vi "TCP_Main.vi"() -> ()   [LabVIEW 2024]
uses:
  <vilib>/Platform/TimedLoop/XDataNode/timing_clust.ctl
  <vilib>/Platform/TimedLoop/XDataNode/nitl_modes.ctl
  <vilib>/Platform/TimedLoop/XDataNode/wakeup.ctl
  <vilib>/addons/Maxon Motor/EPOS2 CANopen/CANopen/sbCANopenBaseClass.lvclass
  <vilib>/platform/TimedLoop/XDataNode/XDataNode.xnode
  <vilib>/Platform/TimedLoop/XDataNode/XDNodeRunTimeDep.lvlib
panel:
  out "TCP Read Error":errorcluster
  out "goal_Tensions":dbl[](array[numeric])
  out "ResetPID":bool
  in  "Motor_index":i32[](array[numeric])=[3, 6, 9, 12, 2, 7, 8, 13, 4, 5, 10, 11, 1, 14]
  out "canERROR":errorcluster[][](array[cluster])
  in  "Control Mode":string="O"
  in  "TARE":bool
  in  "curr_Tensions":dbl[](array[numeric])
  out "DAQ Error":errorcluster
  out "Write Late?":bool
  out "Write Time [us]":i64
  in  "Tare_Tensions":dbl[](array[numeric])=[1.6875269817998764, 0.7228096971601798, 1.962272927280566, 2.6696462364433735, 2.7003690389898463, 3.088938448864716, 1.6430905755314908, 3.0754139877790347, 3.5546581214666455, 3.2737863413382597, 4.727265898547672, 2.6001067118162604, 1.980007529135911, 1.8614502099489874]
  in  "STOP CONTROLLER":bool
  # "\"Error\" codes:\n\n66 - Client Disconnected\n56 - TCP Read time out (every 1ms if no msg comes in)\n0 - packet received"
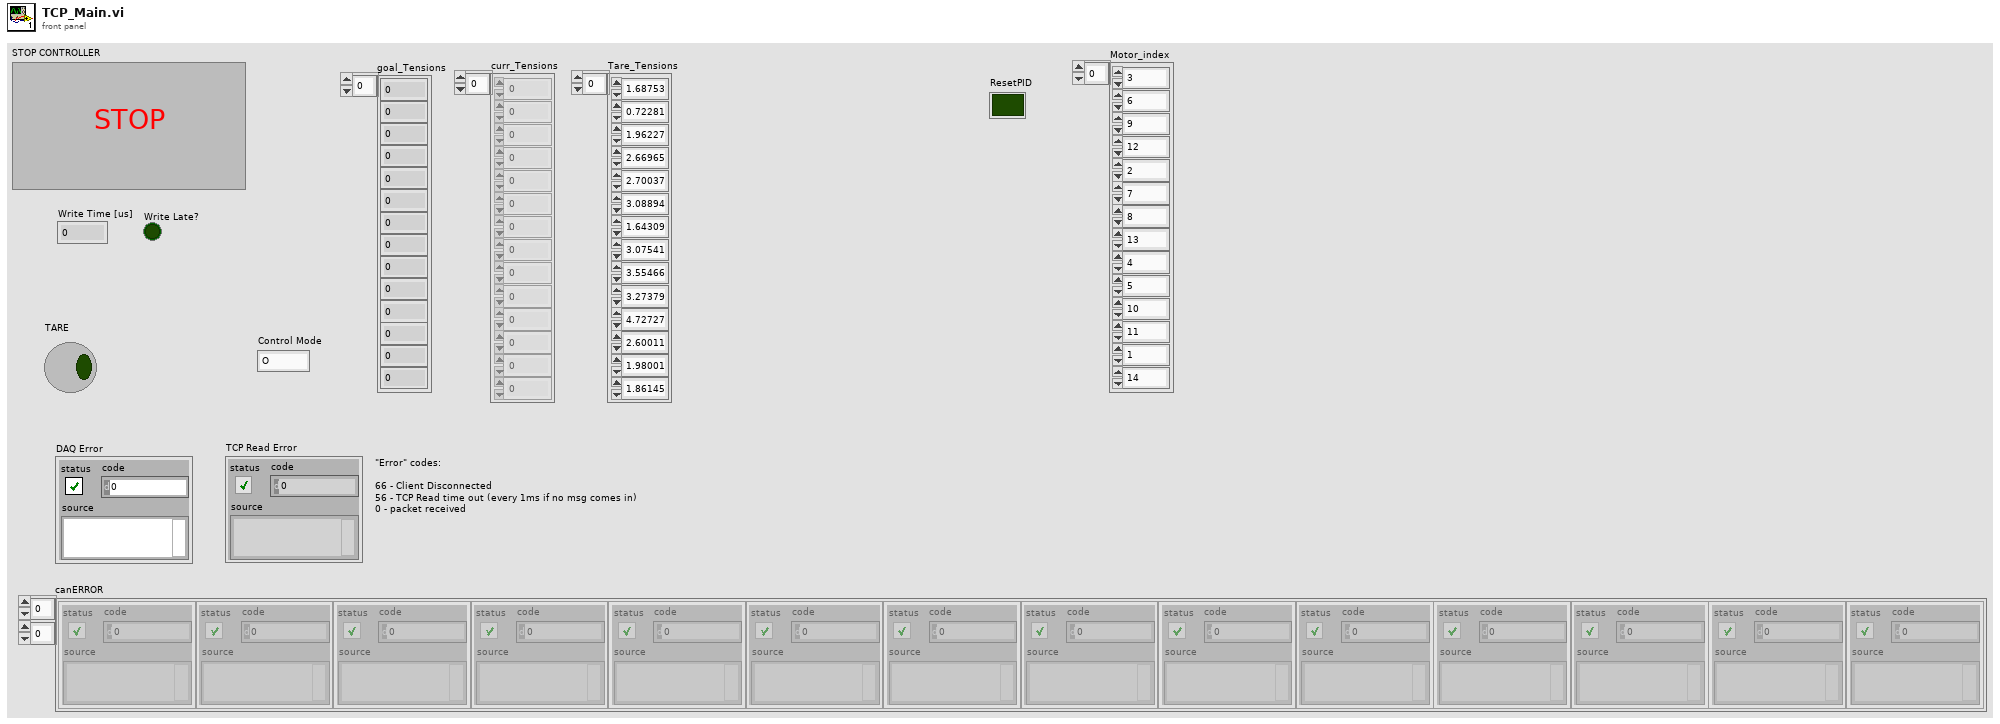
[diagram p1: front panel]
types:
  T1 = enum16{"Standard", "Buffered", "CRLF", "Immediate"}
  T2 = typedef "XDNodeRunTimeDep.lvlib/timing_clust.ctl" = cluster{"Expected End [f-1]":u64, "Actual End [f-1]":u64, "Finished Late? [f-1]":bool, "Expected End [i-1]":u64, "Actual End [i-1]":u64, "Finished Late? [i-1]":bool, "Expected Start [i]":u64, "Actual Start [i]":u64, "Expected Start [f]":u64, "Actual Start [f]":u64, "Source Name":string, "Structure Name":string, "Period":i64, "Deadline":i64, "Offset":i64, "Start":i64, "Priority":i32, "Timeout":i32, "Mode":T3, "Wakeup Reason":T4, "Error":errorcluster, "Source Type":string, "Secondary Source Type":string, "Global End Time":u64, "Global Start Time":u64, "Frame Duration":u64, "Iteration Duration":u64, "Assigned CPU":i32, "I/O Scan Engine Mode":u32}
  T3 = typedef "XDNodeRunTimeDep.lvlib/nitl_modes.ctl" = enum32{"No Change", "Process missed periods, maintain original phase", "Discard missed periods, maintain original phase", "Process missed periods, ignore original phase", "Discard missed periods, ignore original phase"}
  T4 = typedef "XDNodeRunTimeDep.lvlib/wakeup.ctl" = enum32{"Normal", "Aborted", "Asynchronous wakeup", "Timing source error", "Timed loop error", "Timeout"}
  T5 = cluster{"curr_Tensions":dbl[], "goal_Tensions":dbl[]}
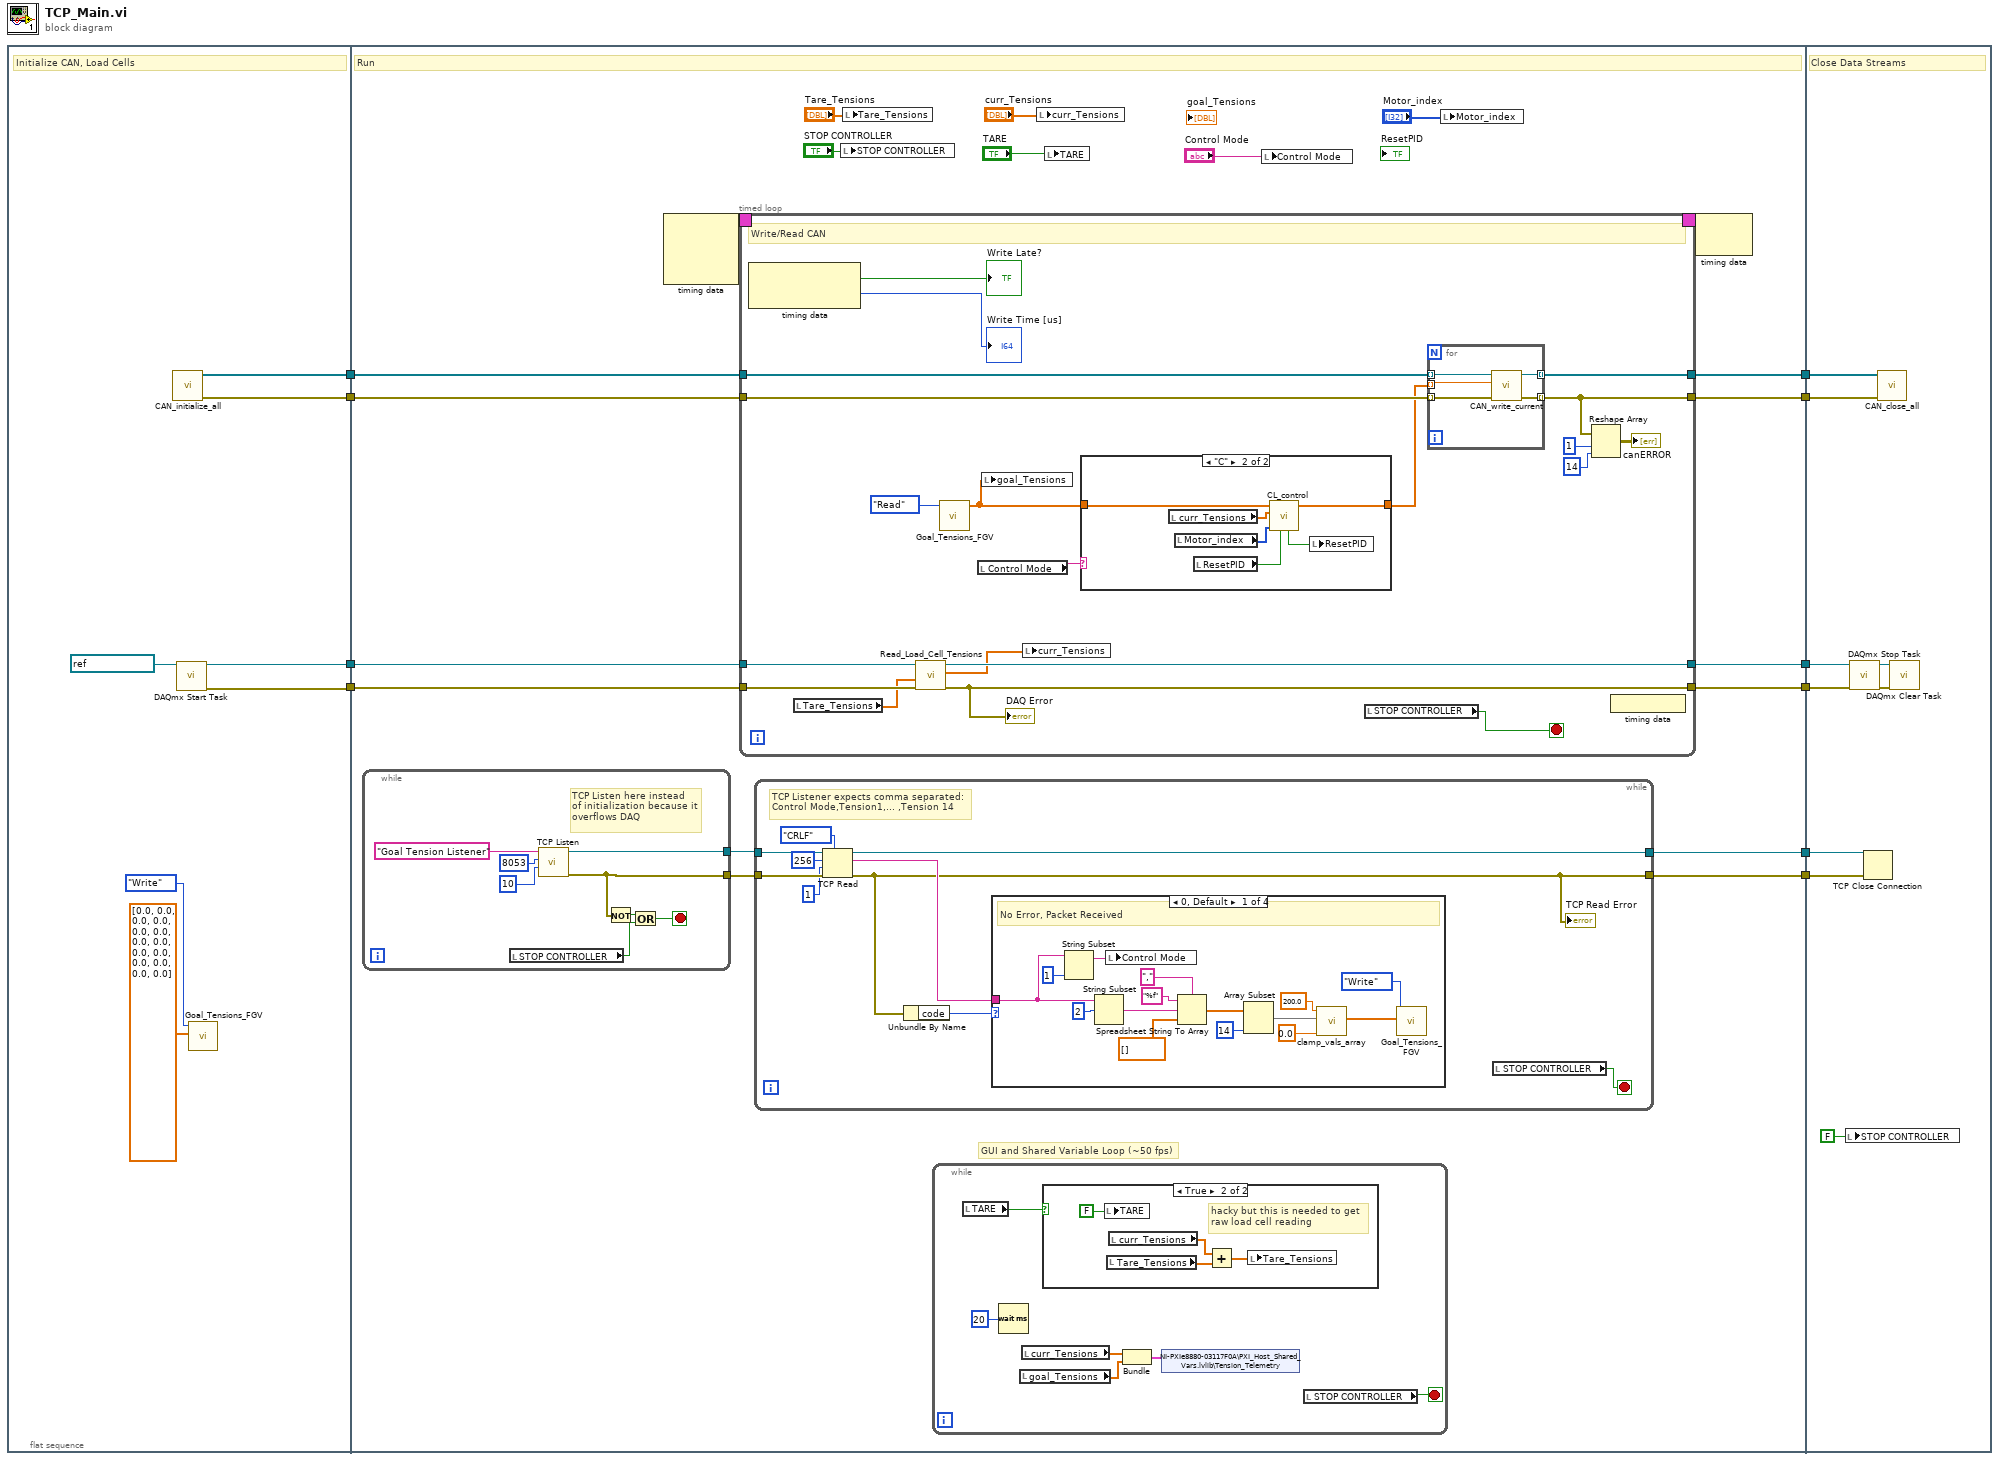
[diagram p0: block diagram]
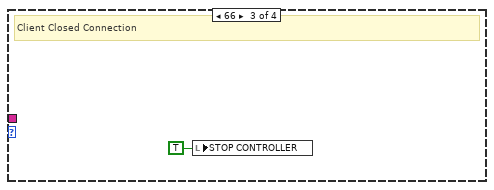
[diagram p3: hidden frame]
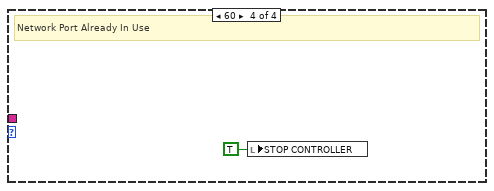
[diagram p4: hidden frame]
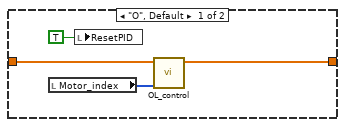
[diagram p6: hidden frame]
diagram:
  n1 = flat-sequence {
    tunnel: [w16] -> w10
    tunnel: [w17] -> w9
    tunnel: [w13] -> w6
    tunnel: [w14] -> w5
    tunnel: w10 -> [w35]
    tunnel: w9 -> [w34]
    tunnel: [w33] -> w8
    tunnel: [w32] -> w7
    tunnel: w6 -> [w30]
    tunnel: w5 -> [w29]
    tunnel: [w28] -> w4
    tunnel: [w27] -> w3
    tunnel: [w20] -> w2
    tunnel: [w21] -> w1
    tunnel: w8 -> [w132]
    tunnel: w7 -> [w131]
    tunnel: w4 -> [w128]
    tunnel: w3 -> [w127]
    tunnel: w2 -> [w125]
    tunnel: w1 -> [w124]
    frame #0 {
      # "Initialize CAN, Load Cells"
      n2 = call "CAN_initialize_all.vi"() -> ("Array of Canopen Sessions"=w17:refnum<class "sbCANopenBaseClass.lvclass">[], "Array of Error out's"=w16:errorcluster[])  [unwired: 5 in]
      n3 = call <vilib>:"DAQmx Start Task.vi"("task/channels in"=refnum<k21> "SCI_TenSen") -> ("task out"=w13:refnum<k21>, "error out"=w14:errorcluster)  [unwired: 13 in]
      n4 = call "Goal_Tensions_FGV.vi"("Write Goal Tension"=dbl[] [0.0, 0.0, 0.0, 0.0, 0.0, 0.0, 0.0, 0.0, 0.0, 0.0, 0.0, 0.0, 0.0, 0.0], "Operation"=enum16{"Write", "Read"}."Write") -> ()  [unwired: 9 in, 1 out]
    }
    frame #1 {
      # "GUI and Shared Variable Loop (~50 fps)"
      # "Run"
      n5 = while {
        tunnel: [w38] -> w19
        tunnel: [w45] -> w18
        stop <- w40 stop-if-true
        # "TCP Listen here instead\nof initialization because it\noverflows DAQ"
        n6 = local read "STOP CONTROLLER"() -> (w41:bool)
        n7 = call <vilib>:"TCP Listen.vi"("timeout ms (wait forever: -1)"=10, "port"=u16 8053, "service name"="Goal Tension Listener") -> ("error out"=w38:errorcluster, "connection ID"=w45:refnum<k5>)  [unwired: 4 in, 3 out]
        n8 = Not(x=w38) -> (.not. x?=w39:bool)
        n9 = Or(x=w39, y=w41) -> (x .or. y?=w40:bool)
      }
      n10 = node-c288() -> (w37:T2)  [unwired: 3 in]
      n11 = timed-loop {
        tunnel: w35 -> [w94]
        tunnel: [w86] -> w33
        timing: w37 -> [_]
        timing-out: [_] -> w36
        tunnel: w34 -> [w95]
        tunnel: [w99] -> w32
        tunnel: w30 -> [w98]
        tunnel: w29 -> [w97]
        tunnel: [w96] -> w28
        tunnel: [w93] -> w27
        stop <- w100 stop-if-true
        # "Write/Read CAN"
        n12 = node-c288() -> (→"Write Late?":bool, →"Write Time [us]":i64)  [unwired: 1 in]
        n13 = local read "Tare_Tensions"() -> (w92:dbl[])
        n14 = call "Read_Load_Cell_Tensions.vi"("error in (no error)"=w97, "Tare Tension"=w92, "Refnum in"=w98) -> ("error out"=w93:errorcluster, "Measured Cable Tensions"=w90:dbl[], "Refnum out"=w96:refnum<k21>)  [unwired: 4 in]
        "DAQ Error" <- w93
        n15 = call "Goal_Tensions_FGV.vi"("Operation"=enum16{"Write", "Read"}."Read") -> ("Read Goal Tension"=w84:dbl[])  [unwired: 10 in]
        n16 = local read "Control Mode"() -> (w91:string)
        n17 = local write "goal_Tensions"(w84) -> ()
        n18 = local write "curr_Tensions"(w90) -> ()
        n19 = case shown="\"C\"" w91 {
          tunnel: [w106 w112] -> w89
          tunnel: w84 -> [w103 w107]
          frame "O", Default {
            n20 = local read "Motor_index"() -> (w105:i32[])
            n21 = local write "ResetPID"(TRUE) -> ()
            n22 = call "OL_control.vi"("Motor_index"=w105, "goal_Tensions"=w103) -> ("can_Current"=w106:dbl[])  [unwired: 9 in]
          }
          frame "C" {
            n23 = local read "curr_Tensions"() -> (w108:dbl[])
            n24 = local read "Motor_index"() -> (w111:i32[])
            n25 = local read "ResetPID"() -> (w110:bool)
            n26 = call "CL_control.vi"("ResetPID"=w110, "Motor_index"=w111, "curr_Tensions"=w108, "goal_Tensions"=w107) -> ("can_Current"=w112:dbl[], "Reset PID (output)"=w109:bool)  [unwired: 6 in]
            n27 = local write "ResetPID"(w109) -> ()
          }
        }
        n28 = local read "STOP CONTROLLER"() -> (w100:bool)
        n29 = for {
          tunnel: [w114] -> w99 mode=indexing
          tunnel: [w115] -> w86 mode=indexing
          tunnel: w95 -> [w117] mode=indexing
          tunnel: w94 -> [w116] mode=indexing
          tunnel: w89 -> [w113] mode=indexing
          n30 = call "CAN_write_current.vi"("error in"=w116, "Current Command [mA]"=w113, "CANopen Session In"=w117) -> ("error out"=w115:errorcluster, "CANopen Session Out"=w114:refnum<class "sbCANopenBaseClass.lvclass">)  [unwired: 7 in]
        }
        n31 = Reshape Array(w86, 1 ("dimension size"), 14 ("dimension size")) -> (→"canERROR":errorcluster[][])
        n32 = node-c288() -> ()  [unwired: 1 out]
      }
      n33 = while {
        tunnel: [w47] -> w20
        tunnel: [w55] -> w21
        tunnel: w19 -> [w53]
        tunnel: w18 -> [w52]
        stop <- w49 stop-if-true
        # "TCP Listener expects comma separated:\nControl Mode,Tension1,... ,Tension 14"
        n34 = TCP Read(connection ID=w52, bytes to read=256, error in (no error)=w53, 7:T1."CRLF" ("mode (standard)"), 9:1 ("timeout ms (25000)")) -> (connection ID out=w55:refnum<k5>, data out=w54:string, error out=w47:errorcluster)
        "TCP Read Error" <- w47
        n35 = Unbundle By Name(w47) -> ("code"=w48:i32)
        n36 = case shown="0, Default" w48 {
          tunnel: w54 -> [w68 _ _ _]
          frame 0, Default {
            # "No Error, Packet Received"
            n37 = String Subset(string=w68, length (rest)=1 ("length (rest)")) -> (substring=w69:string)  [unwired: 1 in]
            n38 = String Subset(string=w68, offset (0)=2) -> (substring=w66:string)  [unwired: 1 in]
            n39 = local write "Control Mode"(w69) -> ()
            n40 = Spreadsheet String To Array(delimiter (Tab)=",", format string="%f", spreadsheet string=w66, array type (2D Dbl)=dbl[] []) -> (array=w61:dbl[])
            n41 = Array Subset(array=w61, length=14) -> (w58:dbl[])  [unwired: 1 in]
            n42 = call "clamp_vals_array.vi"("Min Val"=0.0, "Input Array"=w58, "Max Val"=200.0) -> ("Output Array"=w57:dbl[])  [unwired: 8 in]
            n43 = call "Goal_Tensions_FGV.vi"("Write Goal Tension"=w57, "Operation"=enum16{"Write", "Read"}."Write") -> ()  [unwired: 9 in, 1 out]
          }
          frame 56 {
            # "continue"
            # "Time out Error"
          }
          frame 66 {
            # "Client Closed Connection"
            n44 = local write "STOP CONTROLLER"(TRUE ("STOP CONTROLLER")) -> ()
          }
          frame 60 {
            # "Network Port Already In Use"
            n45 = local write "STOP CONTROLLER"(TRUE ("STOP CONTROLLER")) -> ()
          }
        }
        n46 = local read "STOP CONTROLLER"() -> (w49:bool)
      }
      n47 = local write "STOP CONTROLLER"("STOP CONTROLLER") -> ()
      n48 = local write "Tare_Tensions"("Tare_Tensions") -> ()
      n49 = while {
        stop <- w78 stop-if-true
        n50 = local read "TARE"() -> (w77:bool)
        n51 = Wait (ms)(milliseconds to wait=u32 20) -> ()  [unwired: 1 out]
        n52 = local read "goal_Tensions"() -> (w73:dbl[])
        n53 = local read "curr_Tensions"() -> (w76:dbl[])
        n54 = case shown="True" w77 {
          frame False {
          }
          frame True {
            # "hacky but this is needed to get \nraw load cell reading"
            n55 = local write "TARE"(FALSE ("TARE")) -> ()
            n56 = local read "Tare_Tensions"() -> (w80:dbl[])
            n57 = local read "curr_Tensions"() -> (w81:dbl[])
            n58 = Add(x=w81, y=w80) -> (x+y=w82:dbl[])
            n59 = local write "Tare_Tensions"(w82) -> ()
          }
        }
        n60 = Bundle("curr_Tensions"=w76, "goal_Tensions"=w73) -> (w75:T5)  [unwired: 1 in]
        n61 = shared-variable "NI-PXIe8880-03117F0A\\PXI_Host_Shared_Vars.lvlib\\Tension_Telemetry"(w75) -> ()  [unwired: 1 in, 1 out]
        n62 = local read "STOP CONTROLLER"() -> (w78:bool)
      }
      n63 = local write "curr_Tensions"("curr_Tensions") -> ()
      n64 = local write "TARE"("TARE") -> ()
      n65 = local write "Control Mode"("Control Mode") -> ()
      n66 = local write "Motor_index"("Motor_index") -> ()
      n67 = node-c288(w36) -> ()  [unwired: 1 out]
    }
    frame #2 {
      # "Close Data Streams"
      n68 = local write "STOP CONTROLLER"(FALSE ("STOP CONTROLLER")) -> ()
      n69 = call <vilib>:"DAQmx Stop Task.vi"("task/channels in"=w128, "error in"=w127) -> ("task out"=w129:refnum<k21>, "error out"=w130:errorcluster)  [unwired: 12 in]
      n70 = TCP Close Connection(connection ID=w124, error in (no error)=w125) -> ()  [unwired: 1 in, 2 out]
      n71 = call "CAN_close_all.vi"("Input Error out array"=w132, "Input CANopen Sessions array"=w131) -> ()  [unwired: 10 in]
      n72 = call <vilib>:"DAQmx Clear Task.vi"("task in"=w129, "error in"=w130) -> ()  [unwired: 13 in, 1 out]
    }
  }
